vi "Test exprParser.vi"() -> ()   [LabVIEW 2015]
uses:
  <vilib>/LAVA/AlmostEqual/AlmostEqual_ULPs_DBL.vi
  <vilib>/LAVA/Robust CSV/Robust CSV.lvlib
  <vilib>/LAVA/AlmostEqual/AlmostEqual.lvlib
  <vilib>/gmath/NI_Gmath.lvlib
panel:
  out "Variables":cluster{string, dbl}[](array[cluster]) {"?" format="%_20e"}
  out "NumTests":i32
  out "Failed cases":cluster{string, dbl, "Result":dbl, dbl}[](array[cluster]) {"?" format="%_20e"; "Result" format="%_20e"; "?" format="%_20e"}
  out "NumFails":i32
  in  "Tolerance (ULPs)":u32=100
  out "Test Cases":T1(array[cluster]) {"?" format="%_20e"; "Result" format="%_20e"}
  in  "file path in":path=path "eqTestCases_exprParser.csv"
  # "Notes:"
  # "- euler's number is not pre-defined by formula parser. It will be assigned to variable \"e\""
  # "- comparison operators are not supported"
  # "- exponents are evaluated from left to right (like excel does)"
  # "Expected"
  # "Actual"
  # "Difference"
  # "Expected Result"
  # "Actual Result"
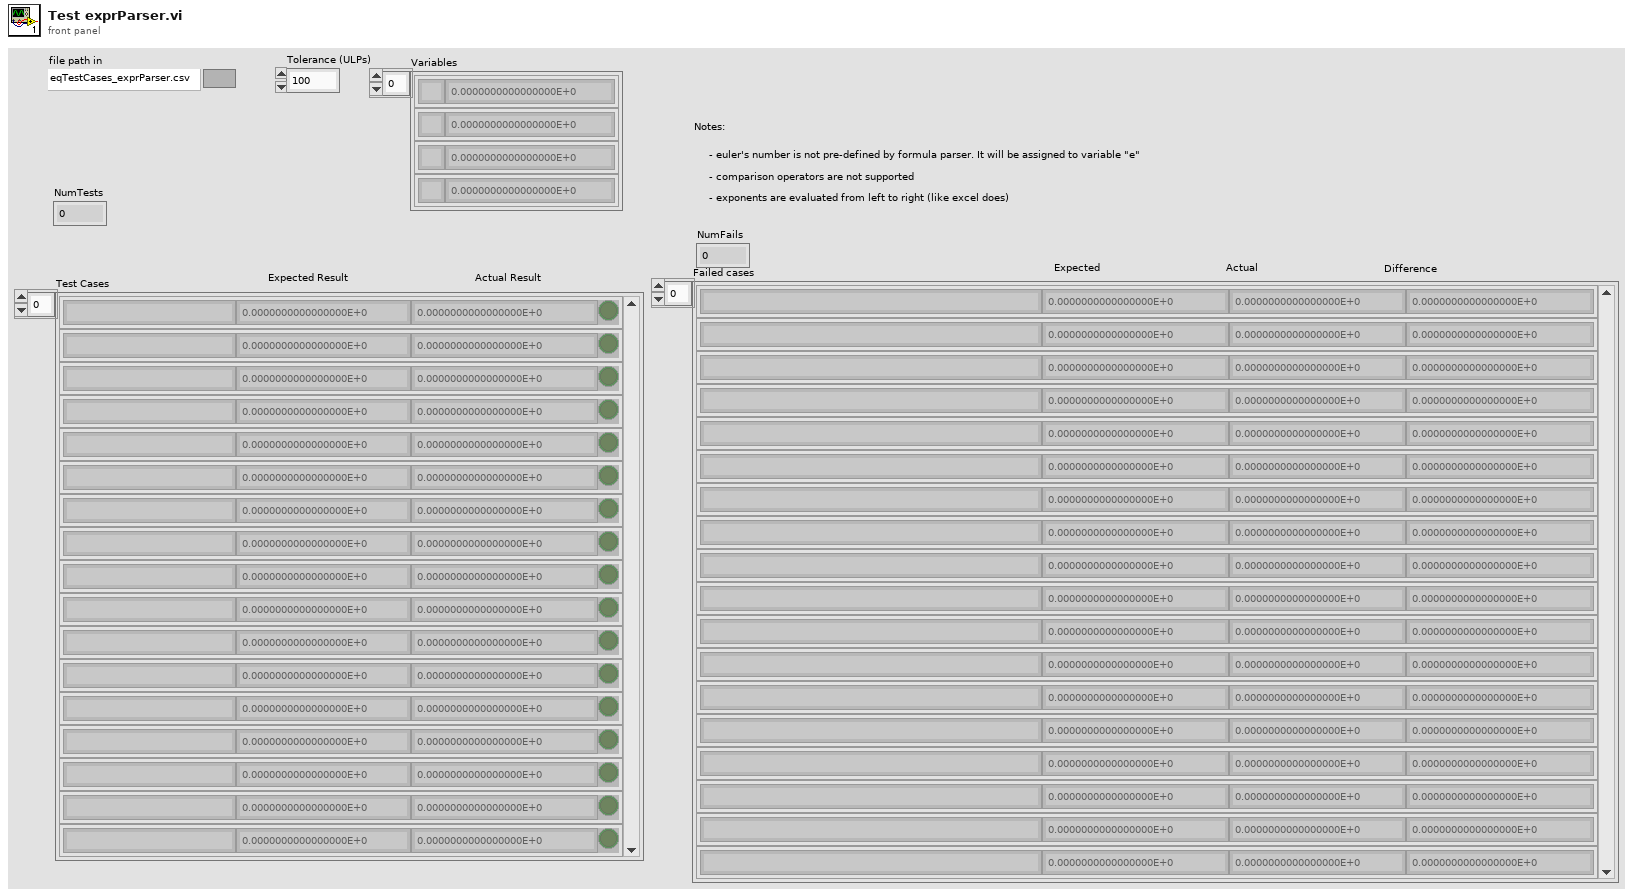
[diagram p1: front panel]
types:
  T1 = cluster{string, dbl, "Result":dbl, "X = Y +/- #ULPs?":bool}[]
  T2 = cluster{string, dbl, "y value":dbl, "X = Y +/- #ULPs?":bool}
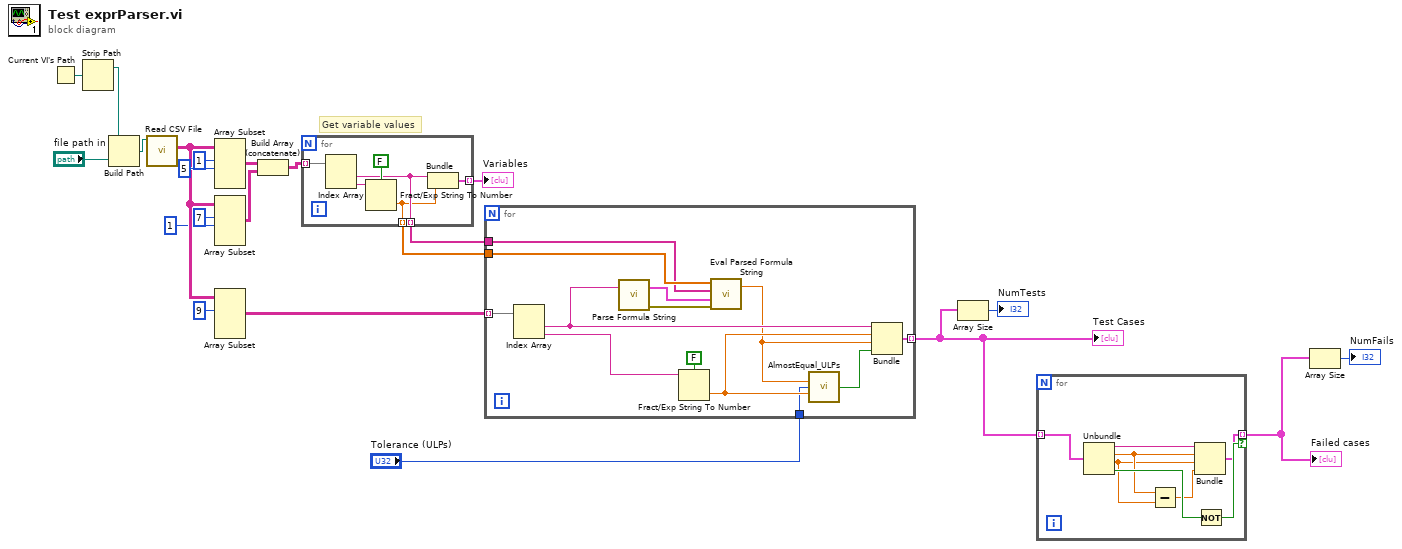
[diagram p0: block diagram]
diagram:
  # "Get variable values"
  n1 = Current VI's Path() -> (path=w10:path)
  n2 = Strip Path(path=w10) -> (stripped path=w8:path)  [unwired: 1 out]
  n3 = Build Path(base path=w8, name or relative path="file path in") -> (appended path=w7:path)
  n4 = call <vilib>:"Read CSV File.vi"("file path in"=w7) -> ("2-D array"=w6:string[][])  [unwired: 8 in, 2 out]
  n5 = Array Subset(array=w6, index (row)=1 ("index"), length (row)=5 ("length")) -> (w3:string[][])  [unwired: 2 in]
  n6 = Array Subset(array=w6, index (row)=7 ("index"), length (row)=1 ("length")) -> (w2:string[][])  [unwired: 2 in]
  n7 = Array Subset(array=w6, index (row)=9 ("index")) -> (w19:string[][])  [unwired: 3 in]
  n8 = Build Array (concatenate)(w3, w2) -> (w1:string[][])
  n9 = for {
    tunnel: w1 -> [w28] mode=indexing
    tunnel: [w25] -> w11 mode=indexing
    tunnel: [w24] -> w13 mode=indexing
    tunnel: [w23] -> w12 mode=indexing
    n10 = Index Array(array=w28) -> (element #1=w24:string, element #2=w27:string)  [unwired: 2 in]
    n11 = Fract/Exp String To Number(use system decimal point (T)=FALSE, string=w27) -> (number=w23:dbl)  [unwired: 2 in, 1 out]
    n12 = Bundle(w24, w23) -> (w25:cluster{string, dbl})  [unwired: 1 in]
  }
  "Variables" <- w11
  n13 = for {
    tunnel: w19 -> [w41] mode=indexing
    tunnel: [w36] -> w15 mode=indexing
    tunnel: "Tolerance (ULPs)" -> [w35]
    tunnel: w13 -> [w30]
    tunnel: w12 -> [w31]
    n14 = Index Array(array=w41) -> (element #1=w32:string, element #2=w39:string)  [unwired: 2 in]
    n15 = call <vilib>:"Parse Formula String.vi"("formula"=w32) -> ("error out"=w34:errorcluster, "Parsed Formula"=w33:cluster{"Table":i32[][], "Y Values":dbl[]})  [unwired: 1 in]
    n16 = Fract/Exp String To Number(use system decimal point (T)=FALSE, string=w39) -> (number=w38:dbl)  [unwired: 2 in, 1 out]
    n17 = call <vilib>:"Eval Parsed Formula String.vi"("error in (no error)"=w34, "Parsed Formula"=w33, "Variables"=w30, "X Values"=w31) -> ("y value"=w29:dbl)  [unwired: 1 out]
    n18 = call-poly <vilib>:"AlmostEqual_ULPs.vi"("X"=w29, "Tolerance (5 ULPs)"=w35, "Y"=w38) -> ("X = Y +/- #ULPs?"=w37:bool)  [unwired: 12 in]
    n19 = Bundle(w32, w38, "y value"=w29, "X = Y +/- #ULPs?"=w37) -> (w36:T2)  [unwired: 1 in]
  }
  "Test Cases" <- w15
  n20 = Array Size(array=w15) -> (size(s)=→"NumTests":i32)
  n21 = for {
    tunnel: w15 -> [w49] mode=indexing
    tunnel: [w42] -> w17 mode=indexing if=w47
    n22 = Unbundle(w49) -> (w46:string, w45:dbl, "y value"=w44:dbl, "X = Y +/- #ULPs?"=w48:bool)
    n23 = Subtract(x=w45, y=w44) -> (x-y=w43:dbl)
    n24 = Bundle(w46, w45, "y value"=w44, w43) -> (w42:cluster{string, dbl, "y value":dbl, dbl})  [unwired: 1 in]
    n25 = Not(x=w48) -> (.not. x?=w47:bool)
  }
  "Failed cases" <- w17
  n26 = Array Size(array=w17) -> (size(s)=→"NumFails":i32)
